vi "VIH UI - Undo Focused Control - Check Focus.vi"(11 "VI Refnum":refnum<vi>) -> (3 "dup VI Refnum":refnum<vi>)   [LabVIEW 2014]
doc: "::: VI Helpeks :::\nCopyright (c) 2000-2026 Konstantin Shifershteyn. All rights reserved."
panel:
  # "VI Helpeks\nCopyright (c) 2012-2026 Konstantin Shifershteyn"
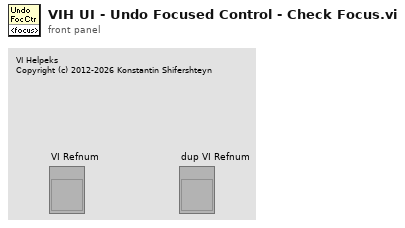
[diagram p1: front panel]
types:
  T1 = cluster{"Ctl Refnum":refnum<vi>, "Ctl Label":string, "Undo Cnt":dbl, "Redo Cnt":dbl}
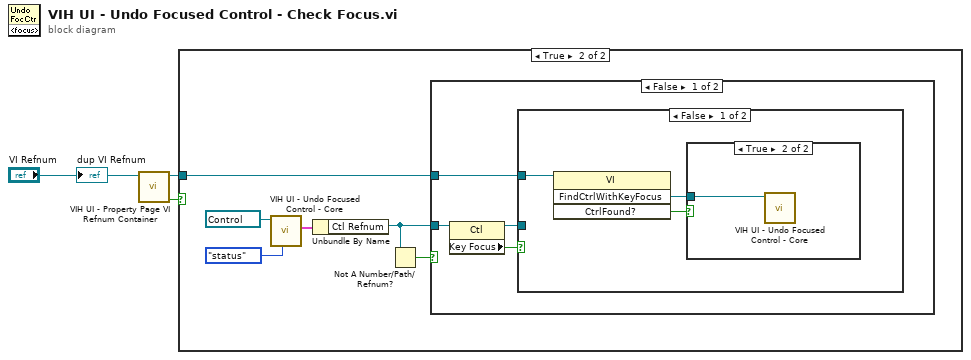
[diagram p0: block diagram]
diagram:
  n1 = call "VIH UI - Property Page VI Refnum Container.vi"("VI Refnum"="VI Refnum") -> ("active"=w3:bool, "VI Refnum out"=w2:refnum<vi>)  [unwired: 9 in]
  n2 = case shown="True" w3 {
    tunnel: w2 -> [_ w4]
    frame False {
    }
    frame True {
      n3 = call "VIH UI - Undo Focused Control - Core.vi"("cmd (save)"=enum16{"Init", "status", "save", "undo", "redo"}."status" ("cmd (click)"), "Ctl Refnum"=refnum<vi> refnum) -> ("Status"=w9:T1)  [unwired: 7 in, 2 out]
      n4 = Unbundle By Name(w9) -> ("Ctl Refnum"=w6:refnum<vi>)
      n5 = Not A Number/Path/Refnum?(number/path/refnum=w6) -> (NaN/Path/Refnum?=w5:bool)
      n6 = case shown="False" w5 {
        tunnel: w4 -> [w12 _]
        tunnel: w6 -> [w11 _]
        frame False {
          n7 = property class="Ctl"(reference=w11) -> (reference out=w10:refnum<vi>, "Key Focus"=w13:bool)  [unwired: 1 in, 1 out]
          n8 = case shown="False" w13 {
            tunnel: w12 -> [w16 _]
            tunnel: w10 -> [_ _]
            frame False {
              n9 = invoke class="VI" method="FindCtrlWithKeyFocus"(reference=w16) -> ("FindCtrlWithKeyFocus"=w15:refnum<vi>, "CtrlFound?"=w14:bool)  [unwired: 3 in, 2 out]
              n10 = case shown="True" w14 {
                tunnel: w15 -> [_ w17]
                frame False {
                }
                frame True {
                  n11 = call "VIH UI - Undo Focused Control - Core.vi"("Ctl Refnum"=w17) -> ()  [unwired: 8 in, 3 out]
                }
              }
            }
            frame True {
            }
          }
        }
        frame True {
        }
      }
    }
  }
  "dup VI Refnum" <- "VI Refnum"
